vi "Lab09_task2_backup2.vi"() -> ()   [LabVIEW 2022 SP3]
uses:
  <vilib>/DAQmx/read.llb/DAQmx Read.vi
  <vilib>/DAQmx/read.llb/DAQmx Read (Analog 1D Wfm NChan NSamp).vi
  <vilib>/Utility/file.llb/Write Delimited Spreadsheet (string).vi
  <vilib>/DAQmx/miscellaneous.llb/DAQmx Fill In Error Info.vi
  <vilib>/measure/mascope.llb/Pulse Measurements N chan.vi
  <vilib>/Utility/file.llb/Write Delimited Spreadsheet (DBL).vi
  <vilib>/measure/NI_MAPro.lvlib
panel:
  out "data":waveform(dbl)[](graph)
  out "Waveform Graph":waveform(dbl)[](graph)
  out "Total execution time (s)":dbl
  in  "reference levels 2":T1={"high ref level"=90.0, "mid ref level"=50.0, "low ref level"=10.0, "ref units"=1} {"ref units" items=["absolute", "percent"]; "high ref level" format="%.2p"; "low ref level" format="%.2p"; "mid ref level" format="%.2p"}
  in  "file path (dialog if empty) 3":path
  out "Time (s) 2":dbl[](array[numeric])
  out "Duty Cycle 2":dbl[](graph)
  out "Period (s) 2":dbl[](graph)
  out "Pulse duration (s) 2":dbl[](graph)
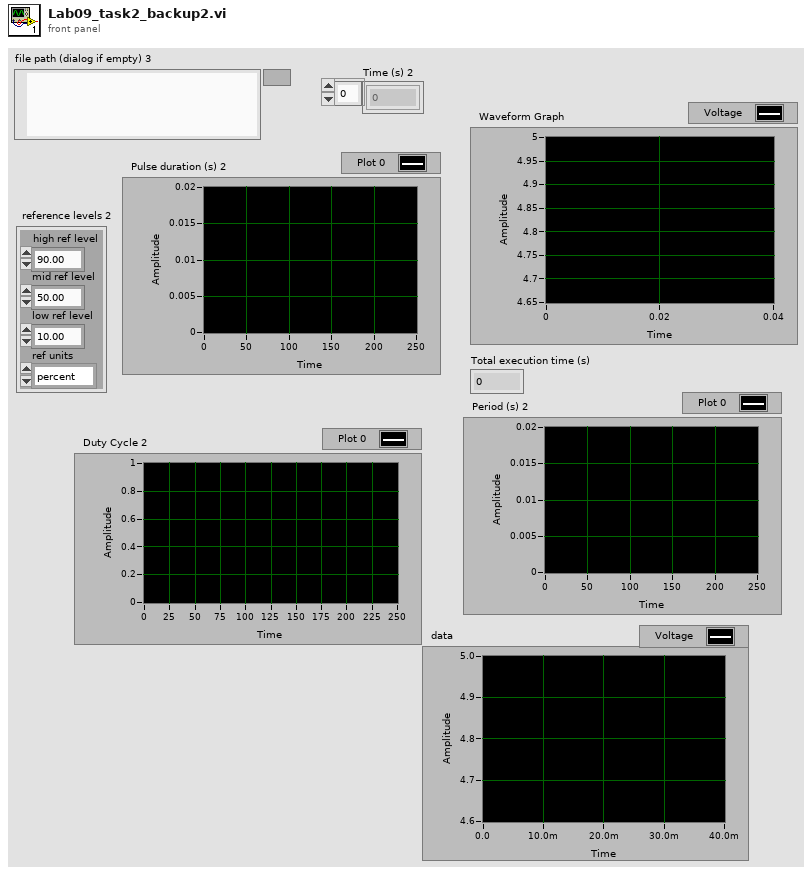
[diagram p1: front panel]
types:
  T1 = cluster{"high ref level":dbl, "mid ref level":dbl, "low ref level":dbl, "ref units":u16}
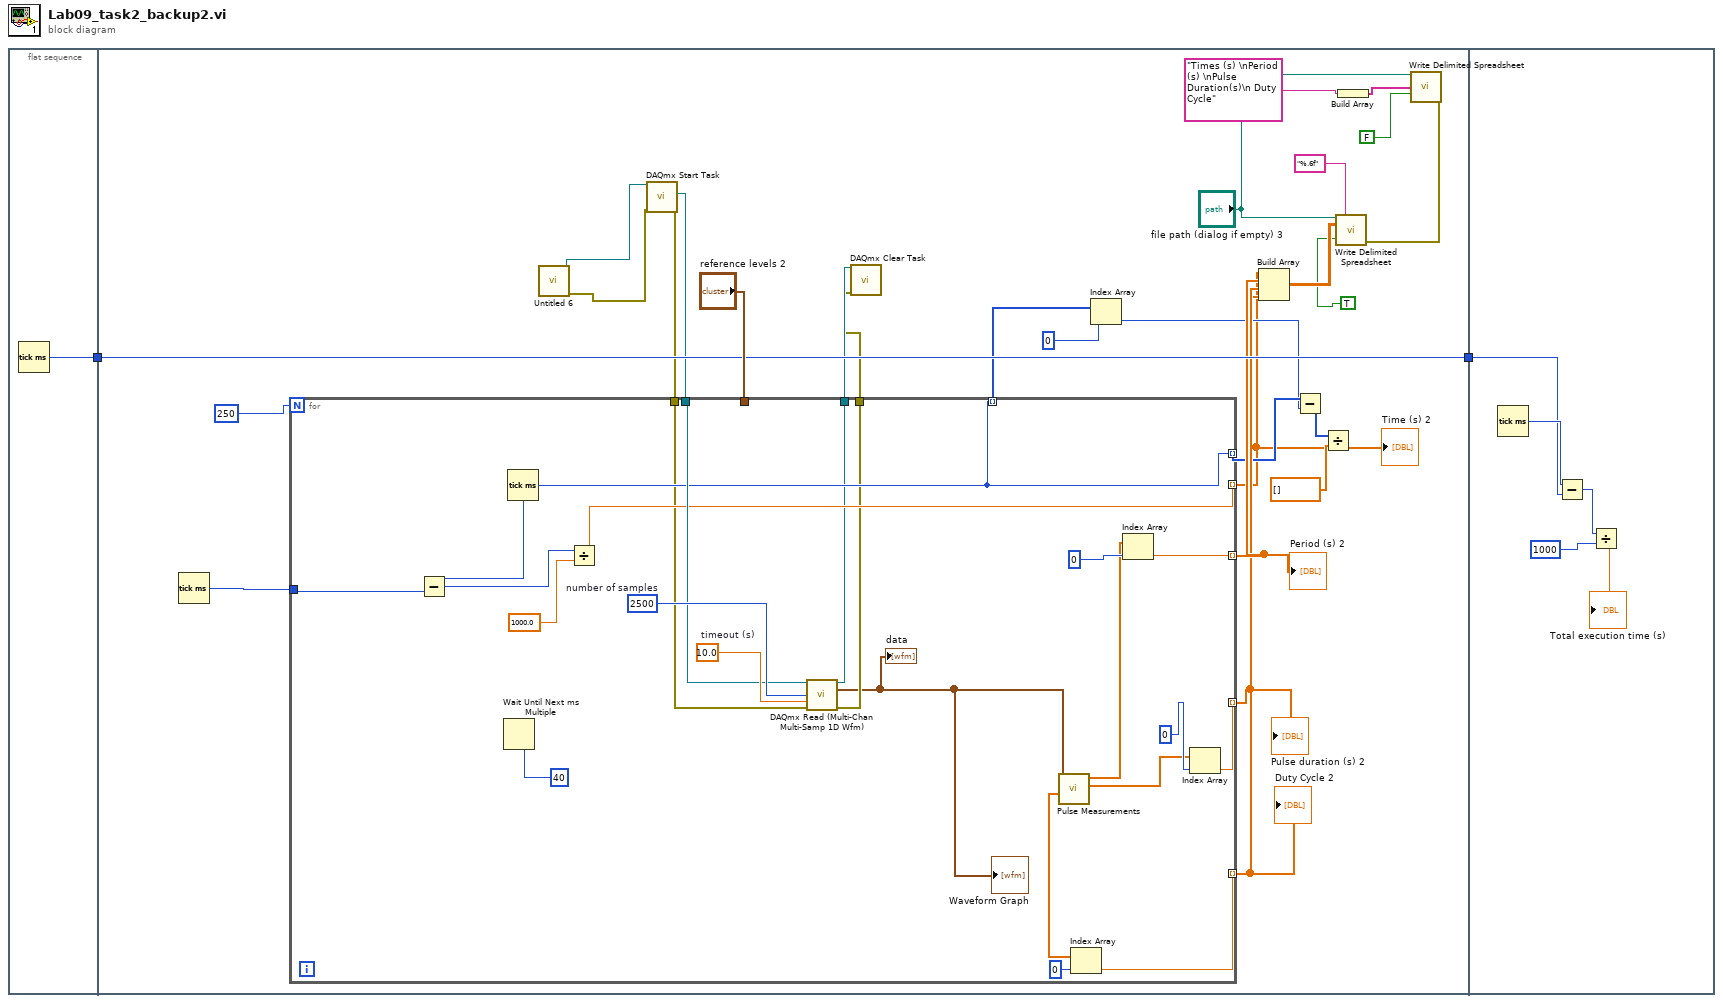
[diagram p0: block diagram]
diagram:
  n1 = flat-sequence {
    tunnel: [w3] -> w2
    tunnel: w2 -> [w23]
    tunnel: [w23] -> w1
    tunnel: w1 -> [w57]
    frame #0 {
      n2 = Tick Count (ms)() -> (millisecond timer value=w3:u32)
    }
    frame #1 {
      n3 = Tick Count (ms)() -> (millisecond timer value=w5:u32)
      n4 = call "Untitled 6.vi"() -> ("error out"=w19:errorcluster, "task out"=w18:refnum<k21>)  [unwired: 10 in]
      n5 = call <vilib>:"DAQmx Start Task.vi"("task/channels in"=w18, "error in"=w19) -> ("task out"=w17:refnum<k21>, "error out"=w16:errorcluster)  [unwired: 12 in]
      n6 = for {
        N: 250 -> [_]
        tunnel: [w47] -> w12 mode=indexing
        tunnel: [w52] -> w11 mode=indexing
        tunnel: [w49] -> w10 mode=indexing
        tunnel: "reference levels 2" -> [_]
        tunnel: [w40] -> w9 mode=indexing
        tunnel: [w33] -> w21
        tunnel: [w35] -> w20
        tunnel: w17 -> [w41]
        tunnel: w16 -> [w34]
        tunnel: [w40] -> w7 mode=indexing
        tunnel: w5 -> [w39]
        tunnel: [w36] -> w4 mode=indexing
        w45 = 10.0  # timeout (s)
        w46 = 2500  # number of samples
        n7 = Wait Until Next ms Multiple(millisecond multiple=u32 40) -> ()  [unwired: 1 out]
        n8 = Tick Count (ms)() -> (millisecond timer value=w40:u32)
        n9 = Subtract(x=w40, y=w39) -> (x-y=w38:u32)
        n10 = Divide(x=w38, y=1000.0) -> (x/y=w36:dbl)
        n11 = call-poly "DAQmx Read (Multi-Chan Multi-Samp 1D Wfm).vi"("task/channels in"=w41, "number of samples per channel"=w46, "timeout"=w45, "error in"=w34) -> ("task out"=w33:refnum<k21>, "data"=w32:waveform(dbl)[], "error out"=w35:errorcluster)  [unwired: 9 in]
        "Waveform Graph" <- w32
        "data" <- w32
        n12 = call-poly <vilib>:"Pulse Measurements.vi"("signal(s) in"=w32) -> ("duty cycle"=w42:dbl[], "pulse duration"=w43:dbl[], "period"=w44:dbl[])  [unwired: 6 in, 2 out]
        n13 = Index Array(array=w42, index=0) -> (element=w49:dbl)
        n14 = Index Array(array=w44, index=0) -> (element=w47:dbl)
        n15 = Index Array(array=w43, index=0) -> (element=w52:dbl)
      }
      "Pulse duration (s) 2" <- w11
      "Period (s) 2" <- w12
      "Duty Cycle 2" <- w10
      "Time (s) 2" <- w4
      n16 = call <vilib>:"DAQmx Clear Task.vi"("task in"=w21, "error in"=w20) -> ()  [unwired: 13 in, 1 out]
      n17 = Index Array(array=w7, index=0) -> (element=w6:u32)
      n18 = Build Array(w4, w12, w11, w10) -> (w29:dbl[][])
      n19 = Subtract(x=w9, y=w6) -> (x-y=w30:u32[])
      n20 = Divide(x=w30, y=dbl[] []) -> ()  [unwired: 1 out]
      n21 = Build Array("Times (s) \nPeriod (s) \nPulse Duration(s)\n Duty Cycle") -> (w26:string[])
      n22 = call-poly <vilib>:"Write Delimited Spreadsheet.vi"("file path (dialog if empty)"="file path (dialog if empty) 3", "1D data"=w26, "append to file? (new file:F)"=FALSE) -> ("error out"=w14:errorcluster)  [unwired: 11 in, 1 out]
      n23 = call-poly <vilib>:"Write Delimited Spreadsheet.vi"("file path (dialog if empty)"="file path (dialog if empty) 3", "format (%.3f)"="%.6f", "2D data"=w29, "error in (no error)"=w14, "transpose? (no:F)"=TRUE) -> ()  [unwired: 9 in, 2 out]
    }
    frame #2 {
      n24 = Tick Count (ms)() -> (millisecond timer value=w58:u32)
      n25 = Subtract(x=w58, y=w57) -> (x-y=w56:u32)
      n26 = Divide(x=w56, y=u32 1000) -> (x/y=→"Total execution time (s)":dbl)
    }
  }
